vi "set Display Line.vi"(8 "error in (no error)":errorcluster, 9 "Line Index":i32, 10 "Amplitude":dbl, 11 "FSV-40N in":refnum<class "FSV-40N.lvclass">) -> (0 "error out":errorcluster, 3 "FSV-40N out":refnum<class "FSV-40N.lvclass">)   [LabVIEW 2023, in "Spectrum Analyzer.lvlib" / "FSV-40N.lvclass"]
uses:
  FSV-40N.lvclass
  FSV-40N.lvclass/FSV-40N.ctl
panel:
  out "결과 문자열":string
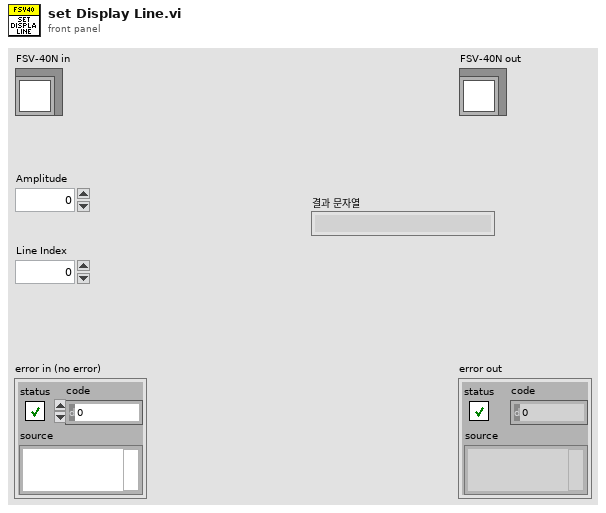
[diagram p1: front panel]
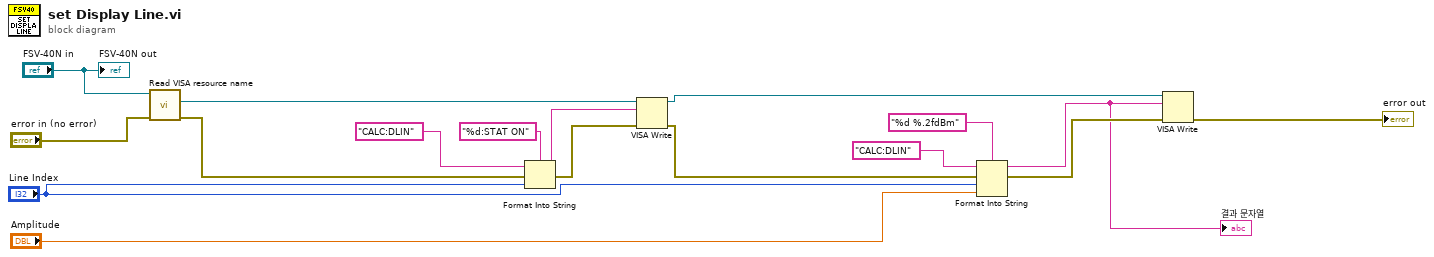
[diagram p0: block diagram]
diagram:
  n1 = call "Read VISA resource name.vi"("error in (no error)"="error in (no error)", "FSV-40N in"="FSV-40N in") -> ("error out"=w8:errorcluster, "VISA resource name"=w6:refnum<visa-resource-name>)  [unwired: 7 in, 1 out]
  n2 = Format Into String(format string="%d:STAT ON" ("포맷 문자열"), initial string="CALC:DLIN", error in=w8, "Line Index") -> (resulting string=w3:string, error out=w7:errorcluster)
  n3 = VISA Write(VISA resource name=w6, write buffer=w3, error in (no error)=w7) -> (VISA resource name out=w1:refnum<visa-resource-name>, error out=w2:errorcluster)  [unwired: 1 out]
  n4 = Format Into String(format string="%d %.2fdBm" ("포맷 문자열"), initial string="CALC:DLIN", error in=w2, "Line Index", "Amplitude") -> (resulting string=w11:string, error out=w12:errorcluster)
  "결과 문자열" <- w11
  n5 = VISA Write(VISA resource name=w1, write buffer=w11, error in (no error)=w12) -> (error out=→"error out":errorcluster)  [unwired: 2 out]
  "FSV-40N out" <- "FSV-40N in"
